vi "Write Boolean Outputs.vi"(8 "error in (no error)":errorcluster, 11 "Modbus in":refnum<class "Modbus.lvclass">) -> (0 "error out":errorcluster, 3 "Modbus out":refnum<class "Modbus.lvclass">)   [LabVIEW 2026, in "Modbus.lvlib" / "Modbus.lvclass"]
uses:
  Modbus.lvclass
  Modbus.lvclass/Modbus.ctl
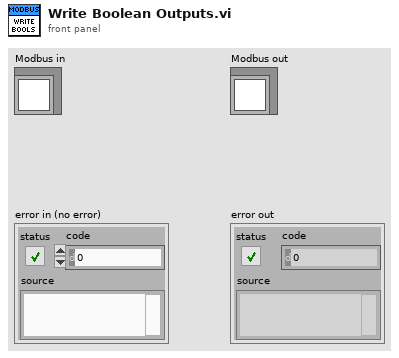
[diagram p1: front panel]
types:
  T1 = typedef "Modbus.lvlib/Modbus.lvclass/Boolean Data.ctl" = cluster{"Channel UID":string, "Valid?":bool, "Table":T2, "Address":i32}
  T2 = typedef "Modbus.lvlib/Modbus.lvclass/Modbus Table.ctl" = enum16{"Discrete Inputs", "Coils", "Input Registers", "Holding Registers"}
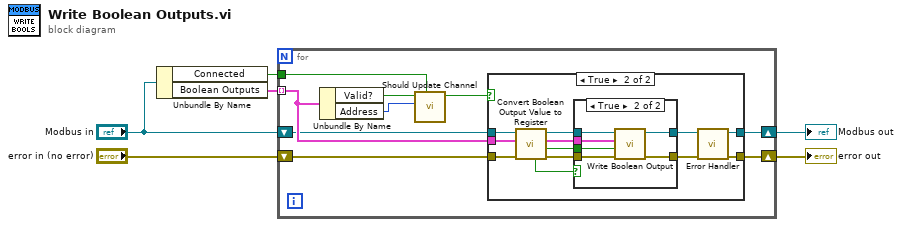
[diagram p0: block diagram]
diagram:
  n1 = Unbundle By Name("Modbus in") -> ("Connected"=w4:bool, "Boolean Outputs"=w6:T1[])
  n2 = for {
    tunnel: w6 -> [w9] mode=indexing
    shift-right: [w11] -> w5
    shift-left: "error in (no error)" -> [w13]
    tunnel: w4 -> [w12]
    shift-right: [w10] -> w3
    shift-left: "Modbus in" -> [w8]
    n3 = Unbundle By Name(w9) -> ("Valid?"=w7:bool, "Address"=w15:i32)
    n4 = call "Should Update Channel.vi"("Connected?"=w12, "Address"=w15, "Valid?"=w7) -> ("Update?"=w14:bool)  [unwired: 8 in]
    n5 = case shown="True" w14 {
      tunnel: [w17 w23] -> w11
      tunnel: w9 -> [_ w28]
      tunnel: w8 -> [w16 w27]
      tunnel: w13 -> [w17 w25]
      tunnel: [w16 w22] -> w10
      frame False {
      }
      frame True {
        n6 = call "Convert Boolean Output Value to Register.vi"("error in (no error)"=w25, "Boolean Output in"=w28, "Plugin in"=w27) -> ("error out"=w29:errorcluster, "Value"=w20:bool, "Boolean Output out"=w26:T1, "Plugin out"=w19:refnum<class "Modbus.lvclass">, "Data Valid"=w21:bool)  [unwired: 4 in]
        n7 = case shown="True" w21 {
          tunnel: [w31 w32] -> w24
          tunnel: w29 -> [w31 w37]
          tunnel: w26 -> [_ w35]
          tunnel: w20 -> [_ w36]
          tunnel: w19 -> [w30 w34]
          tunnel: [w30 w33] -> w18
          frame False {
          }
          frame True {
            n8 = call "Write Boolean Output.vi"("error in (no error)"=w37, "Value"=w36, "Boolean Output"=w35, "Modbus in"=w34) -> ("error out"=w32:errorcluster, "Modbus out"=w33:refnum<class "Modbus.lvclass">)  [unwired: 6 in]
          }
        }
        n9 = call "Error Handler.vi"("error in (no error)"=w24, "Modbus in"=w18) -> ("error out"=w23:errorcluster, "Modbus out"=w22:refnum<class "Modbus.lvclass">)  [unwired: 8 in]
      }
    }
  }
  "Modbus out" <- w3
  "error out" <- w5
